vi "Pre-Build VI - Run Unit Tests.vi"(8 "error in (no error)":errorcluster, 11 "Fail on #todo items":bool) -> (0 "error out":errorcluster, 1 "VIs without test coverage":string[](array[string]), 2 "error type":enum16{"fatal", "non-fatal", "warning"}(ring), 3 "num tests":i32, 4 "VIs not loadable":string[](array[string]), 5 "VIs Failed":string[](array[string]), 6 "VIs with #todo bookmarks":string[](array[string]))   [LabVIEW 2020]
uses:
  <vilib>/addons/_JKI Toolkits/Caraya/Caraya.lvlib
  <vilib>/addons/_JKI Toolkits/Caraya/run-tests/Run Test (Scalar Path).vi
  <vilib>/Utility/miscctls.llb/LVBookmarkInfoTypeDef.ctl
panel:
  out "VIs with #todo's":map{path, T1}(c390)
  out "VIs Succeeded":string[](array[string])
  in  "type specifier VI Refnum (for type only)":refnum<vi>
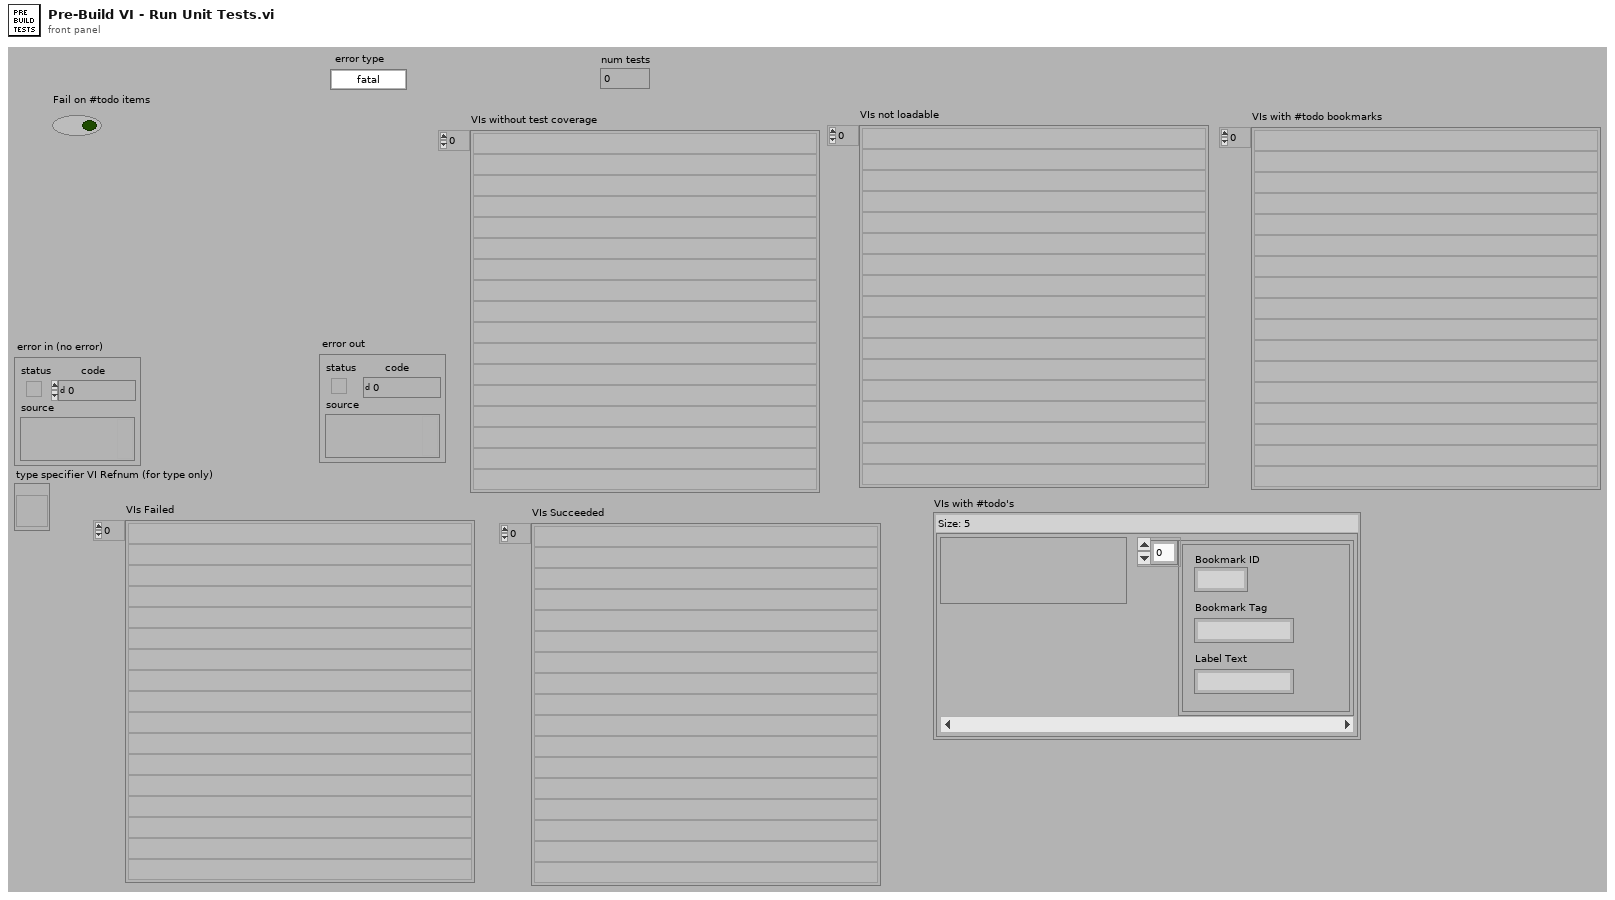
[diagram p1: front panel]
types:
  T1 = typedef "LVBookmarkInfoTypeDef.ctl" = cluster{"Bookmark ID":u32, "Bookmark Tag":string, "Label Text":string}[]
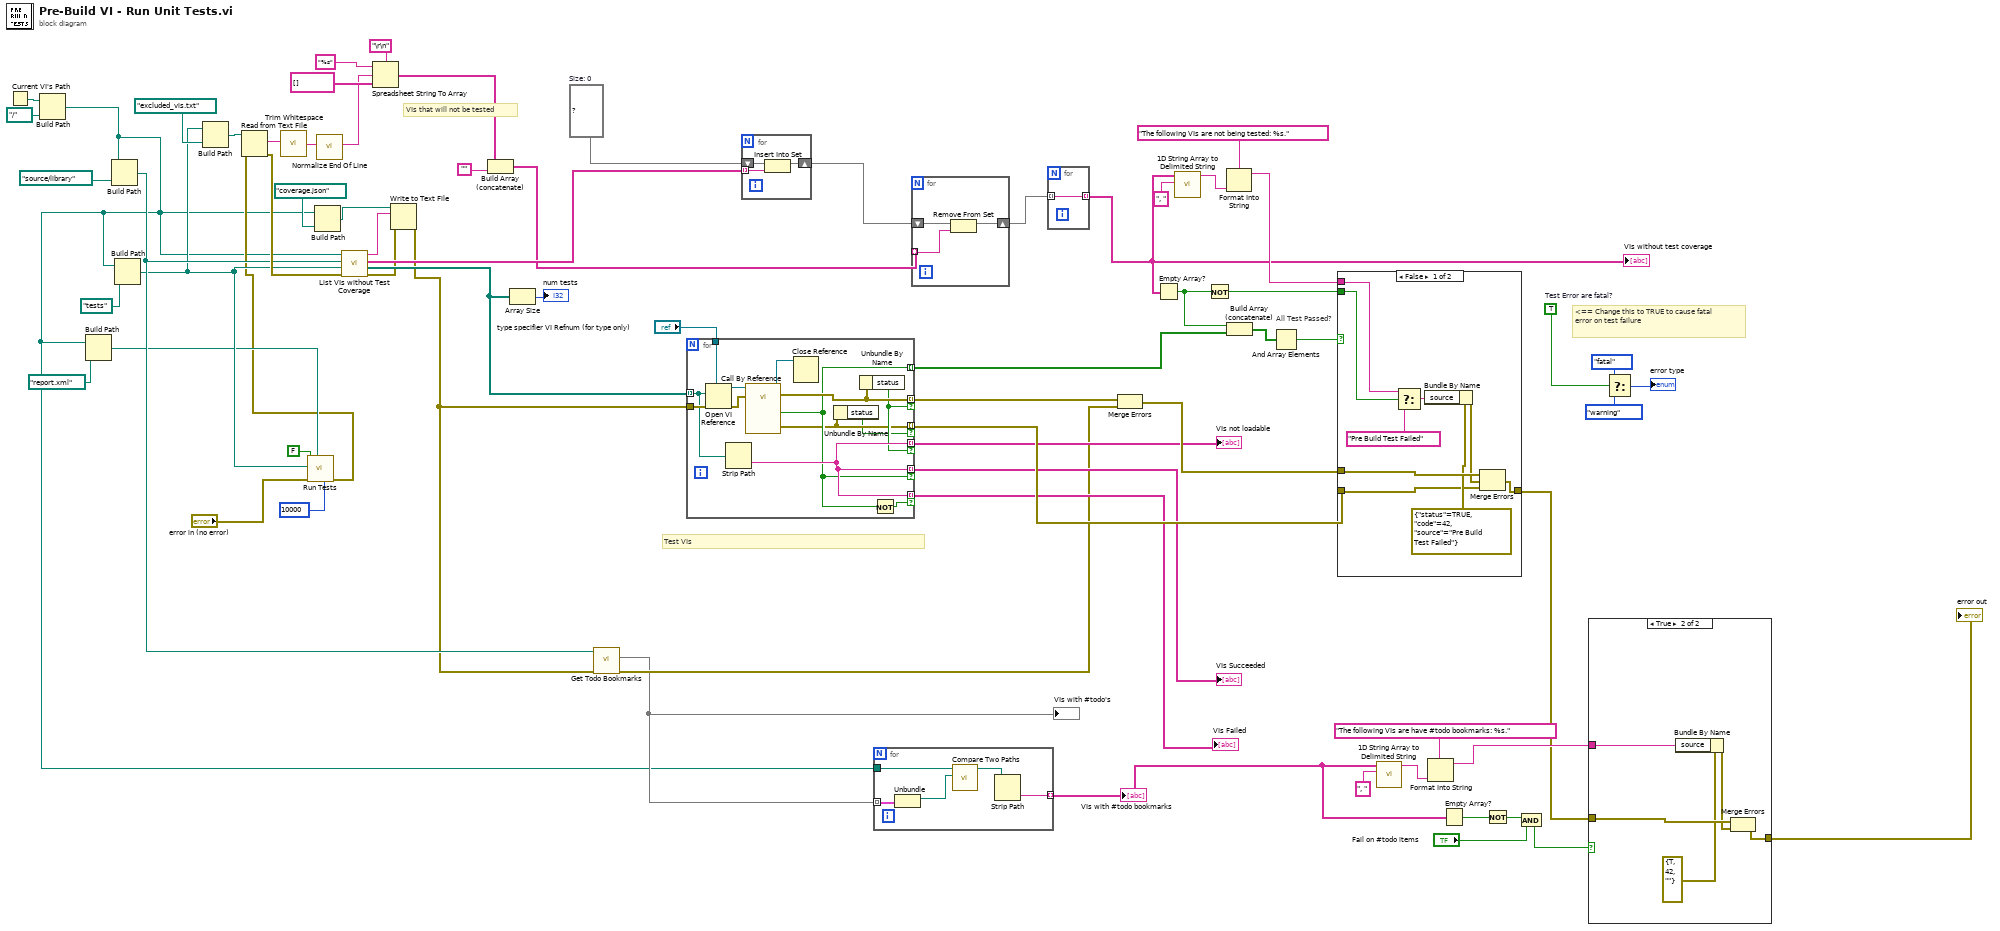
[diagram p0: block diagram]
diagram:
  w44 = set{string} {}  # Size: 0
  w63 = TRUE  # Test Error are fatal?
  # "VIs that will not be tested"
  # "<== Change this to TRUE to cause fatal error on test failure"
  # "All Test Passed?"
  # "Test VIs"
  n1 = Current VI's Path() -> (path=w50:path)
  n2 = Build Path(base path=w50, name or relative path=path "../..") -> (appended path=w1:path)
  n3 = Build Path(base path=w1, name or relative path=path "report.xml" ("Relative path (.)")) -> (appended path=w11:path)
  n4 = Build Path(base path=w1, name or relative path=path "source/library" ("Relative path (.)")) -> (appended path=w28:path)
  n5 = Build Path(base path=w1, name or relative path=path "tests" ("Relative path (.)")) -> (appended path=w14:path)
  n6 = Build Path(base path=w14, name or relative path=path "excluded_vis.txt" ("Relative path (.)")) -> (appended path=w45:path)
  n7 = call-poly <vilib>:"Run Tests.vi"("timeout (2000 ms)"=10000, "Report Path"=w11, "error in"="error in (no error)", "Test Path"=w14, "Interactive (T)"=FALSE) -> ("error out"=w8:errorcluster)  [unwired: 5 in, 1 out]
  n8 = Read from Text File(file (use dialog)=w45, error in=w8) -> (text=w32:string, error out=w31:errorcluster)  [unwired: 2 in, 2 out]
  n9 = call <vilib>:"Trim Whitespace.vi"("string"=w32) -> ("trimmed string"=w34:string)  [unwired: 1 in]
  n10 = Build Path(base path=w1, name or relative path=path "coverage.json" ("Relative path (.)")) -> (appended path=w5:path)
  n11 = call <vilib>:"Normalize End Of Line.vi"("string in"=w34) -> ("string out"=w33:string)  [unwired: 7 in]
  n12 = call "List VIs without Test Coverage.vi"("error in (no error)"=w31, "Tests Root"=w14, "Source Root"=w28, "Project Root"=w1) -> ("error out"=w3:errorcluster, "Test VIs"=w30:path[], "VIs without test coverage"=w43:string[], "coverage.json"=w4:string)  [unwired: 4 in]
  n13 = Spreadsheet String To Array(delimiter (Tab)="\r\n", format string="%s", spreadsheet string=w33, array type (2D Dbl)=string[] [] ("appended array")) -> (array=w35:string[])
  n14 = Write to Text File(file (use dialog)=w5, text=w4, error in=w3) -> (error out=w2:errorcluster)  [unwired: 1 in, 2 out]
  n15 = Build Array (concatenate)(w35, "") -> (w41:string[])
  n16 = Array Size(array=w30) -> (size(s)=→"num tests":i32)
  n17 = call "Get Todo Bookmarks.vi"("error in (no error)"=w2, "Directory to Search"=w28) -> ("error out"=w27:errorcluster, "todo bookmarks"=w18:map{path, T1})  [unwired: 8 in]
  "VIs with #todo's" <- w18
  n18 = for {
    tunnel: w30 -> [w77] mode=indexing
    tunnel: "type specifier VI Refnum (for type only)" -> [w83]
    tunnel: [w75] -> w54 mode=indexing
    tunnel: [w72] -> w58 mode=indexing if=w71
    tunnel: w2 -> [w79]
    tunnel: [w78] -> w55 mode=indexing if=w73
    tunnel: [w76] -> w53 mode=indexing if=w73
    tunnel: [w76] -> w52 mode=indexing if=w75
    tunnel: [w76] -> w51 mode=indexing if=w74
    n19 = Open VI Reference(type specifier VI Refnum (for type only)=w83, vi path=w77, error in (no error)=w79) -> (vi reference=w82:refnum<vi>, error out=w81:errorcluster)  [unwired: 3 in]
    n20 = Strip Path(path=w77) -> (name=w76:string)  [unwired: 1 out]
    n21 = call-by-ref "?"(reference=w82, error in=w81) -> (reference out=w80:refnum<vi>, error out=w78:errorcluster, 0:"error out"=w72:errorcluster, "pass"=w75:bool)  [unwired: 10 in]
    n22 = Close Reference(reference=w80) -> ()  [unwired: 1 in, 1 out]
    n23 = Unbundle By Name(w72) -> ("status"=w71:bool)
    n24 = Unbundle By Name(w78) -> ("status"=w73:bool)
    n25 = Not(x=w75) -> (.not. x?=w74:bool)
  }
  "VIs not loadable" <- w53
  "VIs Succeeded" <- w52
  "VIs Failed" <- w51
  n26 = for {
    tunnel: w43 -> [w86] mode=indexing
    shift-right: [w84] -> w42
    shift-left: w44 -> [w85]
    n27 = Insert Into Set(10:w86, 11:w85) -> (3:w84:set{string})  [unwired: 1 out]
  }
  n28 = for {
    tunnel: w18 -> [w91] mode=indexing
    tunnel: w1 -> [w89]
    tunnel: [w87] -> w21 mode=indexing
    n29 = Unbundle(w91) -> ("key type"=w90:path)  [unwired: 1 out]
    n30 = call <vilib>:"Compare Two Paths.vi"("Path 2"=w90, "Path 1"=w89) -> ("Relative Path from 1 to 2"=w88:path)  [unwired: 6 in, 3 out]
    n31 = Strip Path(path=w88) -> (name=w87:string)  [unwired: 1 out]
  }
  "VIs with #todo bookmarks" <- w21
  n32 = for {
    shift-right: [w92] -> w40
    shift-left: w42 -> [w94]
    tunnel: w41 -> [w93] mode=indexing
    n33 = Remove From Set(10:w93, 11:w94) -> (3:w92:set{string})  [unwired: 1 out]
  }
  n34 = for {
    tunnel: [w95] -> w39 mode=indexing
    tunnel: w40 -> [w95] mode=indexing
  }
  "VIs without test coverage" <- w39
  n35 = Merge Errors(w55, w27) -> (w56:errorcluster)
  n36 = Empty Array?(array=w39) -> (empty?=w65:bool)
  n37 = call <vilib>:"1D String Array to Delimited String.vi"("delimiter"=", " ("delimiter (Tab)"), "string array"=w39) -> ("delimited string"=w68:string)  [unwired: 9 in]
  n38 = Not(x=w65) -> (.not. x?=w64:bool)
  n39 = Format Into String(format string="The following VIs are not being tested: %s.", w68) -> (resulting string=w66:string)  [unwired: 2 in, 1 out]
  n40 = Build Array (concatenate)(w65, w54) -> (w26:bool[])
  n41 = And Array Elements(Boolean array=w26) -> (logical AND=w70:bool)
  n42 = case shown="False" w70 {
    tunnel: w56 -> [w104 w105]
    tunnel: [w103 w105] -> w19
    tunnel: w64 -> [w102 _]
    tunnel: w66 -> [w101 _]
    tunnel: w58 -> [w96 _]
    frame False {
      n43 = Select(t=w101, s=w102, f="Pre Build Test Failed" ("source")) -> (s? t:f=w99:string)
      n44 = Bundle By Name(cluster=errorcluster {"status"=TRUE, "code"=42, "source"="Pre Build Test Failed"} ("error out"), "source"=w99) -> (w98:errorcluster)
      n45 = Merge Errors(w104, w98, w96) -> (w103:errorcluster)
    }
    frame True {
    }
  }
  n46 = call <vilib>:"1D String Array to Delimited String.vi"("delimiter"=", " ("delimiter (Tab)"), "string array"=w21) -> ("delimited string"=w24:string)  [unwired: 9 in]
  n47 = Format Into String(format string="The following VIs are have #todo bookmarks: %s.", w24) -> (resulting string=w22:string)  [unwired: 2 in, 1 out]
  n48 = Empty Array?(array=w21) -> (empty?=w20:bool)
  n49 = Not(x=w20) -> (.not. x?=w17:bool)
  n50 = And(x=w17, y="Fail on #todo items") -> (x .and. y?=w16:bool)
  n51 = case shown="True" w16 {
    tunnel: w19 -> [w106 w111]
    tunnel: [w106 w107] -> w7
    tunnel: w22 -> [_ w108]
    frame False {
    }
    frame True {
      n52 = Bundle By Name(cluster=errorcluster {"status"=TRUE, "code"=42, "source"=""} ("error out"), "source"=w108) -> (w110:errorcluster)
      n53 = Merge Errors(w111, w110) -> (w107:errorcluster)
    }
  }
  "error out" <- w7
  n54 = Select(t=enum16{"fatal", "non-fatal", "warning"}."fatal" ("error type"), s=w63, f=enum16{"fatal", "non-fatal", "warning"}."warning" ("error type")) -> (s? t:f=→"error type":enum16{"fatal", "non-fatal", "warning"})
